vi "LinearSystemSim_UpdateY.vi"(8 "MeasurementStdDev":T1, 9 "ClampedU":T1, 10 "X":T1, 11 "Linearsystem":T2) -> (0 "Error":bool, 3 "Y":T1)   [LabVIEW 2019, in "Trajectory_Library.lvlib"]
doc: "Updates the Y matrix of the system.\n \nInputs:\n - LinearSystem -- Data cluster\n - currentX -- The current state estimate.\n - ClampedU -- The system inputs (usually voltage).\n - MeasurementStdDev -- Standard deviation vector matrix for measurements\n\nOutputs:\n - Y -- The new Y matrix.\n - Error -- If TRUE, an error occured."
uses:
  Trajectory_Library.lvlib
  <vilib>/Analysis/Matrix/NI_Matrix.lvlib
  <vilib>/Analysis/Matrix/Numeric/Add/Add - RM,RM.vi
  TypeDef/LINEAR_SYSTEM.ctl
  <vilib>/Analysis/Matrix/Datatypes/RealMatrix.ctl
panel:
  # "<States,States>"
  # "<States,Inputs>"
  # "<Outputs,States>"
  # "<Outputs,Inputs>"
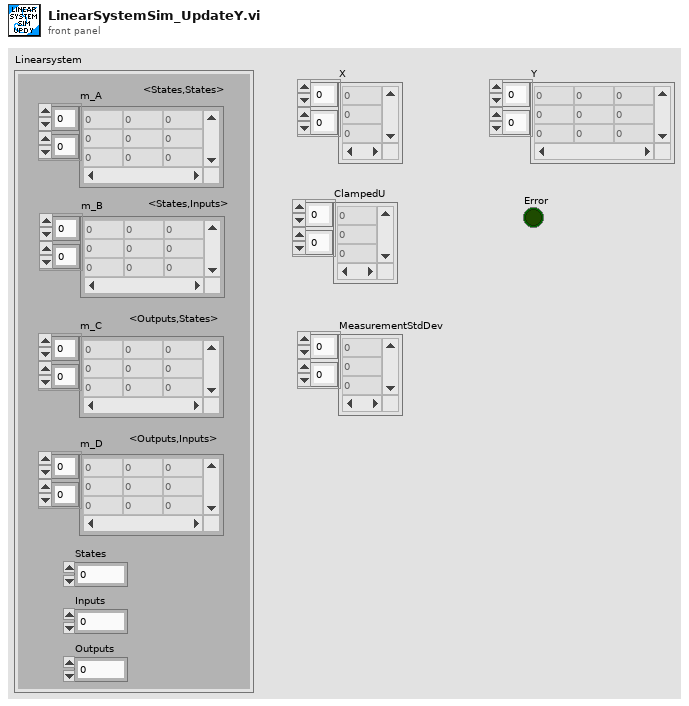
[diagram p1: front panel]
types:
  T1 = typedef "NI_Matrix.lvlib/RealMatrix.ctl" = dbl[][]
  T2 = typedef "Trajectory_Library.lvlib/LINEAR_SYSTEM.ctl" = cluster{"m_A":T1, "m_B":T1, "m_C":T1, "m_D":T1, "States":i32, "Inputs":i32, "Outputs":i32}
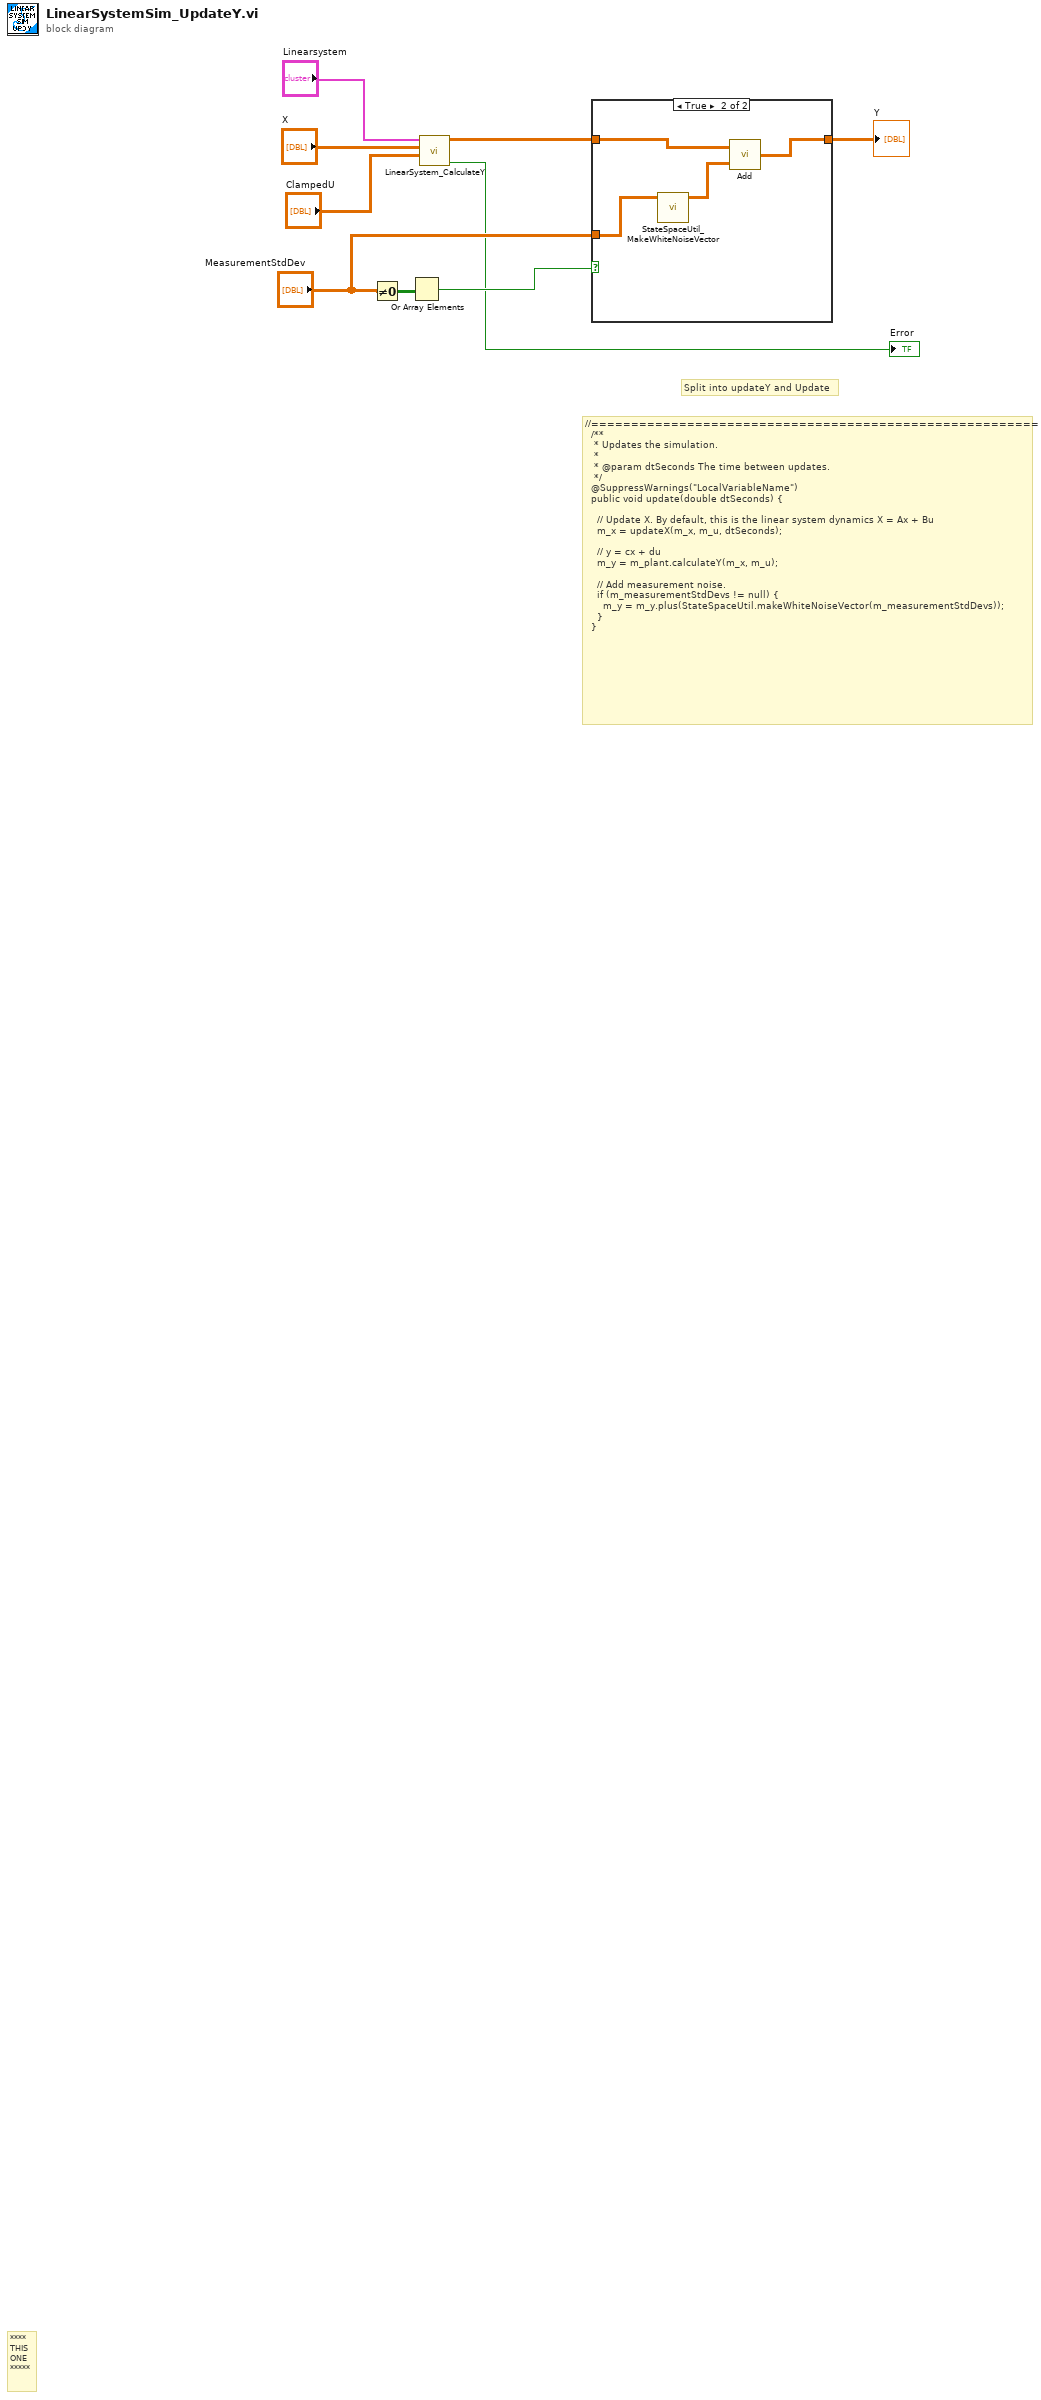
[diagram p0: block diagram]
diagram:
  # "Split into updateY and Update"
  # "//========================================================\n  /**\n   * Updates the simulation.\n   *\n   * @param dtSeconds The time between updates.\n   */\n  @SuppressWarnings(\"LocalVariableName\")\n  public void update(double dtSeconds) {\n\n    // Update X. By default, this is the linear system dynamics X = Ax + Bu\n    m_x = updateX(m_x, m_u, dtSeconds);\n\n    // y = cx + du\n    m_y = m_plant.calculateY(m_x, m_u);\n\n    // Add measurement noise.\n    if (m_measurementStdDevs != null) {\n      m_y = m_y.plus(StateSpaceUtil.makeWhiteNoiseVector(m_measurementStdDevs));\n    }\n  }"
  # "****\nTHIS\nONE\n*****"
  n1 = Not Equal To 0?(x="MeasurementStdDev") -> (x != 0?=w4:bool[][])
  n2 = Or Array Elements(Boolean array=w4) -> (logical OR=w3:bool)
  n3 = call "LinearSystem_CalculateY.vi"("ClampedU"="ClampedU", "X"="X", "Linearsystem"="Linearsystem") -> ("Error"=→"Error":bool, "outY"=w9:T1)  [unwired: 7 in]
  n4 = case shown="True" w3 {
    tunnel: w9 -> [w10 w13]
    tunnel: [w10 w12] -> w6
    tunnel: "MeasurementStdDev" -> [_ w14]
    frame False {
      # "No Noise"
    }
    frame True {
      n5 = call "StateSpaceUtil_MakeWhiteNoiseVector.vi"("StdDevs"=w14) -> ("WhiteNoise"=w11:T1)  [unwired: 9 in, 1 out]
      n6 = call-poly <vilib>:"Add.vi"("Real Matrix B"=w11, "Real Matrix A"=w13) -> ("A + B"=w12:T1)
    }
  }
  "Y" <- w6
